vi "Delete.vi"(8 "error in":errorcluster, 10 "Path":path, 11 "File Manager in":refnum<class "File Manager.lvclass">) -> (0 "error out":errorcluster, 3 "File Manager out":refnum<class "File Manager.lvclass">)   [LabVIEW 2026, in "File Manager.lvclass"]
doc: "Delete a file or folder without prompts."
uses:
  File Manager.lvclass
  File Manager.lvclass/File Manager.ctl
  Interfaces/ILogger/ILogger Messages/Log Msg/Log Msg.lvclass/Log Msg.ctl
  <vilib>/ActorFramework/Message Enqueuer/Message Enqueuer.lvclass/Message Enqueuer.ctl
  <vilib>/ActorFramework/Message Enqueuer/Enqueue.vi
  Interfaces/ILogger/ILogger Messages/Log Msg/Log Msg.lvclass
  C:/Program Files/National Instruments/LabVIEW 2026/vi.lib/ActorFramework/Message/Message.lvclass
  <vilib>/ActorFramework/Message Priority Queue/Priority Enqueue.vi
  <userlib>/_OpenG.lib/file/file.llb/openg_file.lvlib
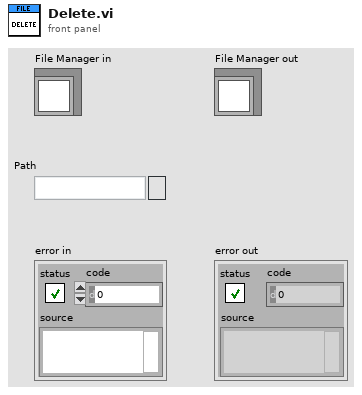
[diagram p1: front panel]
types:
  T1 = typedef "Log Entry--cluster.ctl" = cluster{"Time":timestamp, "Message":string}
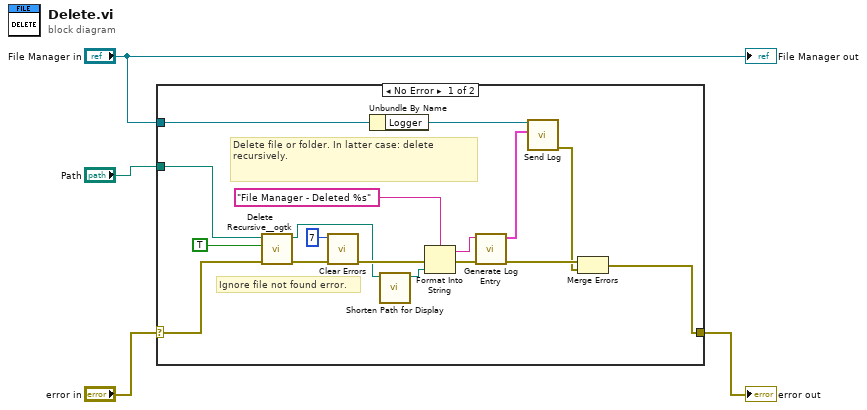
[diagram p0: block diagram]
diagram:
  n1 = case shown="No Error" "error in" {
    selector: "error in" -> [w15 w22]
    tunnel: [w19 w22] -> w4
    tunnel: "Path" -> [w14 _]
    tunnel: "File Manager in" -> [w11 _]
    frame No Error {
      # "Ignore file not found error."
      # "Delete file or folder. In latter case: delete recursively."
      n2 = call <userlib>:"Delete Recursive__ogtk.vi"("error in (no error)"=w15, "Recursive? (FALSE)"=TRUE ("entire hierarchy (F)"), "Path"=w14) -> ("error out"=w17:errorcluster, "dup Path"=w7:path)  [unwired: 7 in]
      n3 = call <vilib>:"Clear Errors.vi"("error in (no error)"=w17, "specific error code to clear (0: all)"=7) -> ("error out"=w16:errorcluster)  [unwired: 4 in, 1 out]
      n4 = Unbundle By Name(w11) -> ("Logger"=w12:refnum<class "Message Enqueuer.lvclass">)
      n5 = call "Shorten Path for Display.vi"("Path"=w7) -> ("Shortened Path"=w6:path)  [unwired: 10 in]
      n6 = Format Into String(format string="File Manager - Deleted %s" ("Message"), error in=w16, w6) -> (resulting string=w9:string, error out=w21:errorcluster)  [unwired: 1 in]
      n7 = call "Generate Log Entry.vi"("error in"=w21, "Message"=w9) -> ("error out"=w20:errorcluster, "Log Entry"=w8:T1)  [unwired: 8 in]
      n8 = call "Send Log.vi"("Log Entry"=w8, "Message Enqueuer"=w12) -> ("error out"=w18:errorcluster)  [unwired: 8 in, 1 out]
      n9 = Merge Errors(w20, w18) -> (w19:errorcluster)
    }
    frame Error {
      # "Pass error without further action."
    }
  }
  "error out" <- w4
  "File Manager out" <- "File Manager in"
